vi "Set Logger Enqueuer.vi"(8 "error in":errorcluster, 10 "Logger":refnum<class "Message Enqueuer.lvclass">, 11 "Runner in":refnum<class "Runner.lvclass">) -> (0 "error out":errorcluster, 3 "Runner out":refnum<class "Runner.lvclass">)   [LabVIEW 2026, in "Runner.lvlib" / "Runner.lvclass"]
doc: "Set the logger enqueuer for a Logger Client."
uses:
  Runner.lvclass
  <vilib>/ActorFramework/Message Enqueuer/Message Enqueuer.lvclass
  Runner.lvclass/Runner.ctl
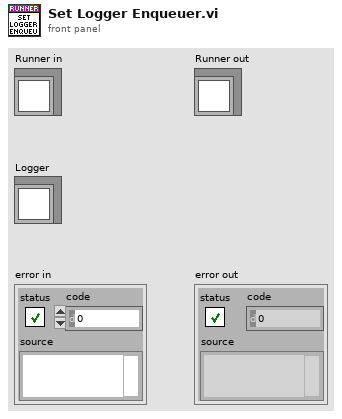
[diagram p1: front panel]
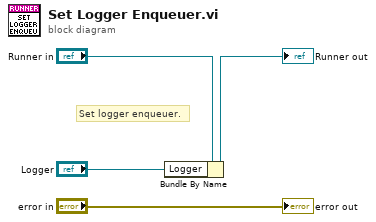
[diagram p0: block diagram]
diagram:
  # "Set logger enqueuer."
  n1 = Bundle By Name(cluster="Runner in", "Logger"="Logger") -> (→"Runner out":refnum<class "Runner.lvclass">)
  "error out" <- "error in"
